vi "query Marker Frequency Count Value.vi"(8 "error in (no error)":errorcluster, 10 "Marker Index":i32=1 min=1, 11 "Keysight 9020A in":refnum<class "Keysight 9020A.lvclass">) -> (0 "error out":errorcluster, 2 "Marker Value":T1 {"X-axis" format="%#_6p"}, 3 "Keysight 9020A out":refnum<class "Keysight 9020A.lvclass">)   [LabVIEW 2023, in "Spectrum Analyzer.lvlib" / "Keysight 9020A.lvclass"]
uses:
  Keysight 9020A.lvclass
  TYPE DEFINITION/TYPE Marker Value.ctl
  Keysight 9020A.lvclass/Keysight 9020A.ctl
  Spectrum Analyzer.lvlib
  <vilib>/ErrorRing/Error Ring.xnode
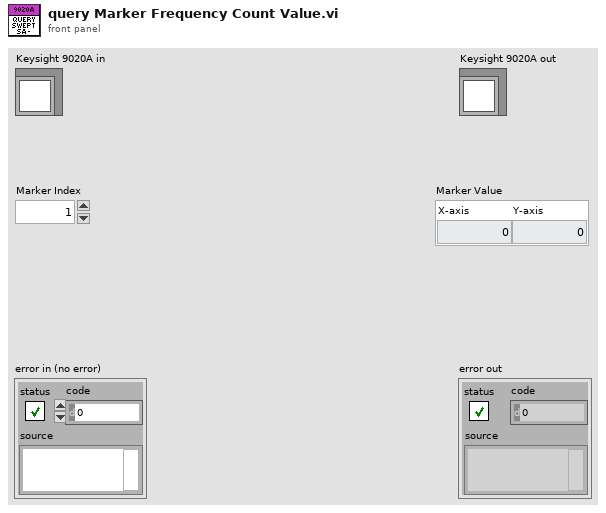
[diagram p1: front panel]
types:
  T1 = typedef "Spectrum Analyzer.lvlib/TYPE Marker Value.ctl" = cluster{"X-axis":dbl, "Y-axis":dbl}
  T2 = typedef "Spectrum Analyzer.lvlib/TYPE Measurement Preset.ctl" = enum16{"Sweep SA Mode", "Channel Power", "Occupied BW", "ACP", "Spurious Emission", "Spurious Emission Mask", "Burst Power (Transmit Power)"}
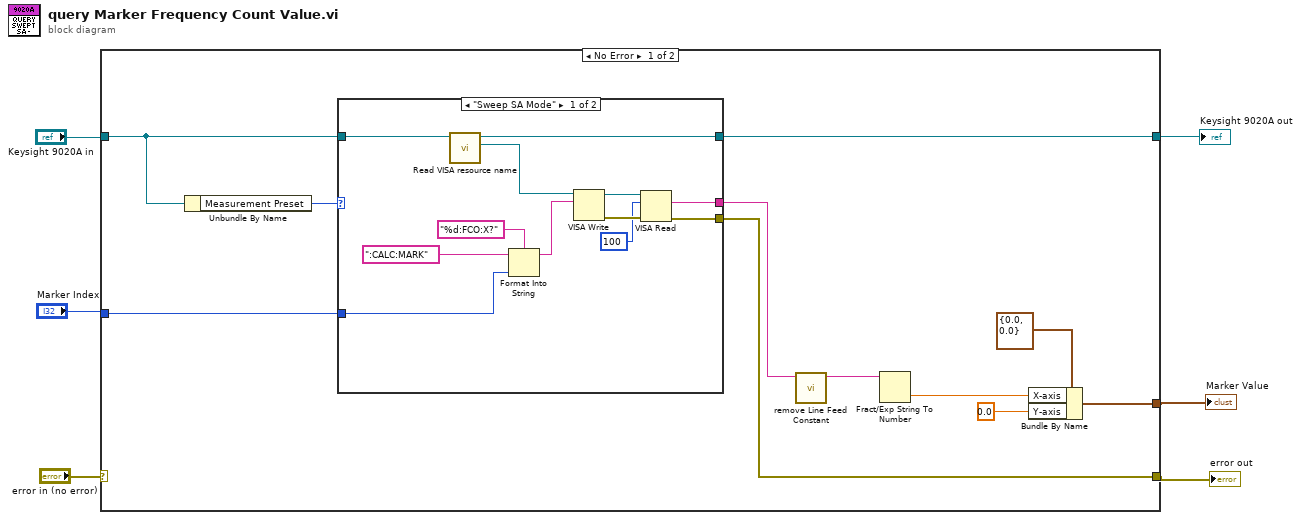
[diagram p0: block diagram]
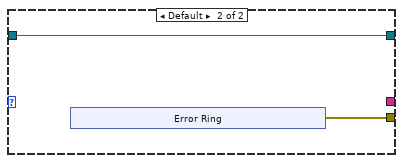
[diagram p2: hidden frame]
diagram:
  n1 = case shown="No Error" "error in (no error)" {
    selector: "error in (no error)" -> [_ w33]
    tunnel: "Keysight 9020A in" -> [w8 w34]
    tunnel: [w17 w34] -> w5
    tunnel: [w9 w33] -> w3
    tunnel: [w13 _] -> w1
    tunnel: "Marker Index" -> [w11 _]
    frame No Error {
      n2 = Unbundle By Name(w8) -> ("Measurement Preset"=w7:T2)
      n3 = case shown="\"Sweep SA Mode\"" w7 {
        tunnel: [w29 w31] -> w17
        tunnel: [w25 _] -> w16
        tunnel: w11 -> [w21 _]
        tunnel: [w20 w30] -> w9
        tunnel: w8 -> [w18 w31]
        frame "Sweep SA Mode" {
          n4 = call "Read VISA resource name.vi"("Keysight 9020A in"=w18) -> ("VISA resource name"=w24:refnum<visa-resource-name>, "Keysight 9020A out"=w29:refnum<class "Keysight 9020A.lvclass">)  [unwired: 8 in, 1 out]
          n5 = Format Into String(format string="%d:FCO:X?", initial string=":CALC:MARK", w21) -> (resulting string=w22:string)  [unwired: 1 in, 1 out]
          n6 = VISA Write(VISA resource name=w24, write buffer=w22) -> (VISA resource name out=w28:refnum<visa-resource-name>, error out=w27:errorcluster)  [unwired: 1 in, 1 out]
          n7 = VISA Read(VISA resource name=w28, byte count=u32 100, error in (no error)=w27) -> (read buffer=w25:string, error out=w20:errorcluster)  [unwired: 2 out]
        }
        frame Default {
          n8 = xnode "Error Ring"() -> ("error out"=w30:errorcluster)
        }
      }
      n9 = call "remove Line Feed Constant.vi"("Input String"=w16) -> ("Line Feed Removed String"=w15:string)  [unwired: 10 in]
      n10 = Fract/Exp String To Number(string=w15) -> (number=w14:dbl)  [unwired: 3 in, 1 out]
      n11 = Bundle By Name(cluster=T1 {"X-axis"=0.0, "Y-axis"=0.0} ("Marker Value 2"), "X-axis"=w14, "Y-axis"=0.0) -> (w13:T1)
    }
    frame Error {
    }
  }
  "error out" <- w3
  "Keysight 9020A out" <- w5
  "Marker Value" <- w1
